vi "Load Config.vi"(8 "error in (no error)":errorcluster) -> (0 "error out":errorcluster, 3 "Array":T3(array[cluster]))   [LabVIEW 2019, in "LINX.lvlib" / "LINX.lvclass"]
uses:
  LINX.lvclass
  LINX Control Shortcut.ctl
  LINX Channel Type.ctl
  LINX Command Message.ctl
  <vilib>/Utility/config.llb/Read Key (String).vi
  <vilib>/Utility/config.llb/Read Key (I32).vi
  <vilib>/Utility/config.llb/NI_LVConfig.lvlib
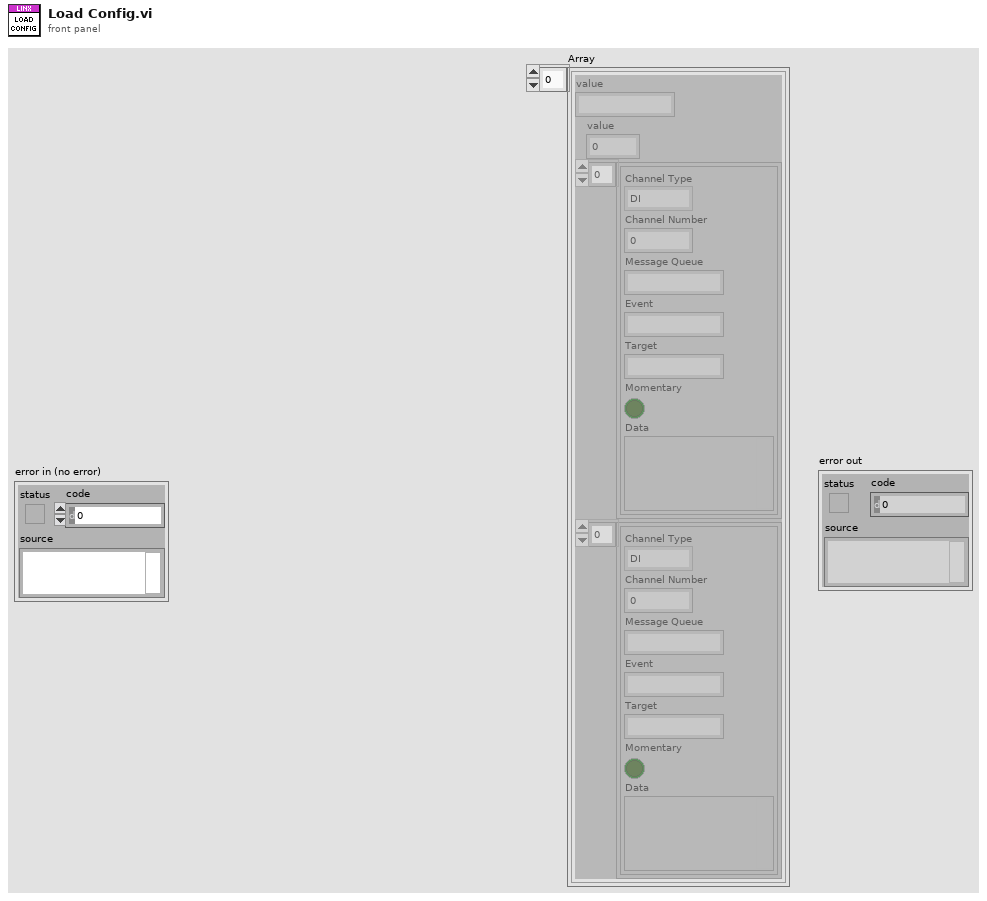
[diagram p1: front panel]
types:
  T1 = typedef "LINX.lvlib/LINX.lvclass/LINX Control Shortcut.ctl" = cluster{"Channel Type":T2, "Channel Number":u8, "Message Queue":string, "Event":string, "Target":string, "Momentary":bool, "Data":variant}
  T2 = typedef "LINX.lvlib/LINX.lvclass/LINX Channel Type.ctl" = enum16{"DI", "AI"}
  T3 = cluster{"value":string, "value":i32, T1[], T1[]}[]
  T4 = typedef "NI_LVConfig.lvlib/Config Data RefNum.ctl" = refnum<k1>
  T5 = typedef "LINX.lvlib/LINX.lvclass/LINX Command Message.ctl" = cluster{"Command":string, "Message Queue":string, "Event":string, "Target":string, "Momentary":bool, "Data":variant}
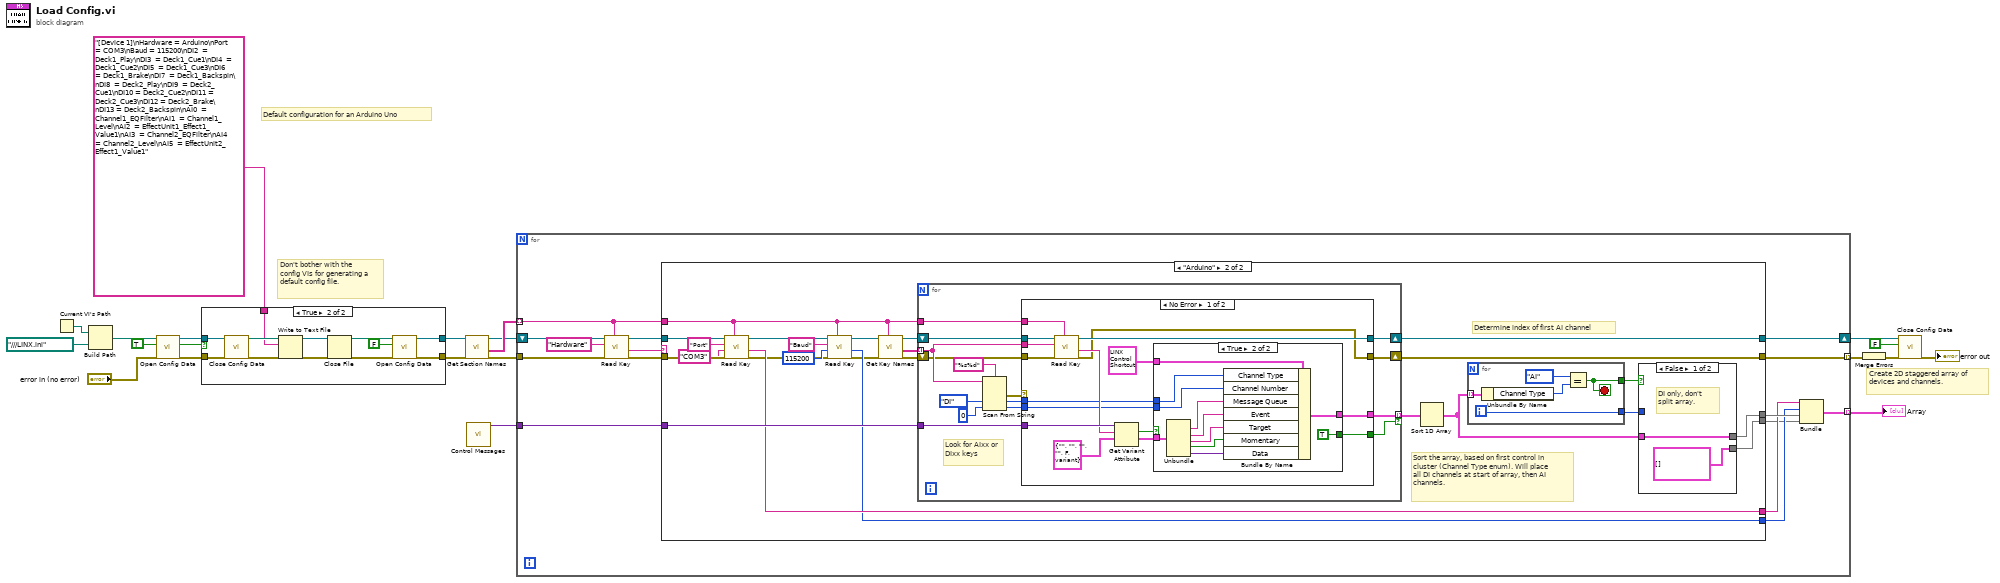
[diagram p0: block diagram]
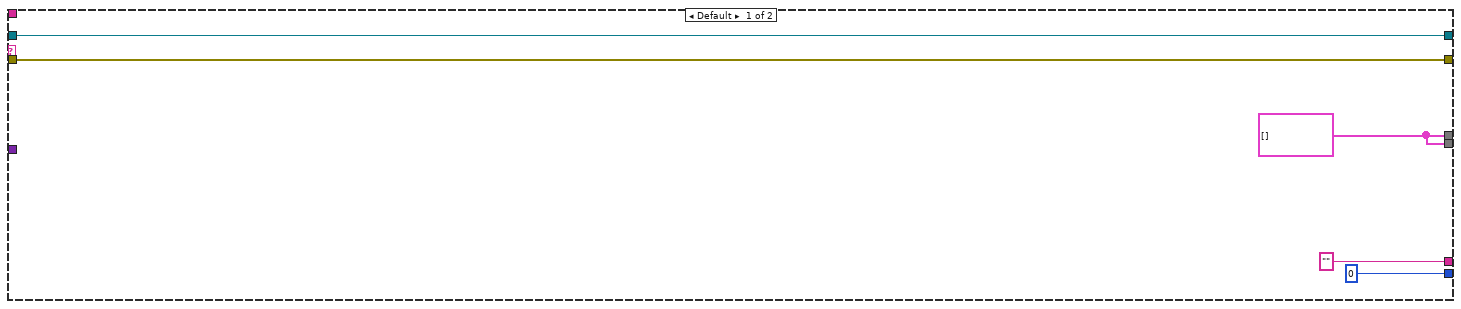
[diagram p3: hidden frame]
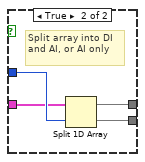
[diagram p4: hidden frame]
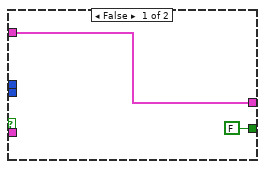
[diagram p5: hidden frame]
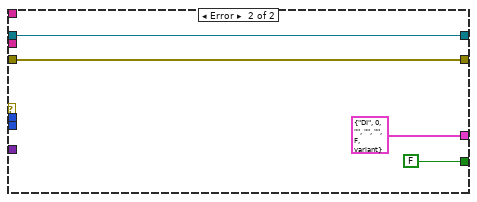
[diagram p6: hidden frame]
diagram:
  # "Don't bother with the config VIs for generating a default config file."
  # "Create 2D staggered array of devices and channels."
  # "Default configuration for an Arduino Uno"
  n1 = Current VI's Path() -> (path=w13:path)
  n2 = Build Path(base path=w13, name or relative path=path "../../../LINX.ini" ("configuration file path")) -> (appended path=w11:path)
  n3 = call <vilib>:"Open Config Data.vi"("error in (no error)"="error in (no error)", "create file if necessary (T)"=TRUE, "configuration file path"=w11) -> ("error out"=w6:errorcluster, "file created?"=w10:bool, "refnum"=w9:T4)  [unwired: 6 in]
  n4 = case shown="True" w10 {
    tunnel: w9 -> [w23 w35]
    tunnel: [w23 w24] -> w8
    tunnel: [w22 w25] -> w7
    tunnel: w6 -> [w22 w34]
    tunnel: "[Device 1]\nHardware = Arduino\nPort = COM3\nBaud = 115200\nDI2  = Deck1_Play\nDI3  = Deck1_Cue1\nDI4  = Deck1_Cue2\nDI5  = Deck1_Cue3\nDI6  = Deck1_Brake\nDI7  = Deck1_Backspin\nDI8  = Deck2_Play\nDI9  = Deck2_Cue1\nDI10 = Deck2_Cue2\nDI11 = Deck2_Cue3\nDI12 = Deck2_Brake\nDI13 = Deck2_Backspin\nAI0  = Channel1_EQFilter\nAI1  = Channel1_Level\nAI2  = EffectUnit1_Effect1_Value1\nAI3  = Channel2_EQFilter\nAI4  = Channel2_Level\nAI5  = EffectUnit2_Effect1_Value1" -> [_ w32]
    frame False {
    }
    frame True {
      n5 = call <vilib>:"Close Config Data.vi"("error in (no error)"=w34, "refnum"=w35) -> ("error out"=w31:errorcluster, "file path"=w33:path)  [unwired: 8 in]
      n6 = Write to Text File(file (use dialog)=w33, text=w32, error in=w31) -> (refnum out=w30:refnum<file>, error out=w29:errorcluster)  [unwired: 1 in, 1 out]
      n7 = Close File(refnum=w30, error in=w29) -> (path=w28:path, error out=w26:errorcluster)
      n8 = call <vilib>:"Open Config Data.vi"("error in (no error)"=w26, "create file if necessary (T)"=FALSE, "configuration file path"=w28) -> ("error out"=w25:errorcluster, "refnum"=w24:T4)  [unwired: 6 in, 1 out]
    }
  }
  n9 = call <vilib>:"Get Section Names.vi"("error in (no error)"=w7, "refnum"=w8) -> ("error out"=w17:errorcluster, "section names"=w19:string[], "refnum out"=w18:T4)  [unwired: 7 in]
  n10 = call "Control Messages.vi"() -> ("Shortcuts"=w20:variant)  [unwired: 11 in]
  n11 = for {
    tunnel: w19 -> [w46] mode=indexing
    tunnel: w17 -> [w38]
    shift-right: [w44] -> w15
    shift-left: w18 -> [w50]
    tunnel: w20 -> [w45]
    tunnel: [w42] -> w16 mode=indexing
    tunnel: [w36] -> w2 mode=indexing
    n12 = call-poly <vilib>:"Read Key.vi"("section"=w46, "error in (no error)"=w38, "key"="Hardware", "refnum"=w50) -> ("error out"=w37:errorcluster, "value"=w48:string, "refnum out"=w47:T4)  [unwired: 4 in, 1 out]
    n13 = case shown="\"Arduino\"" w48 {
      tunnel: w47 -> [w55 w80]
      tunnel: w46 -> [_ w73]
      tunnel: w45 -> [_ w72]
      tunnel: [w55 w70] -> w44
      tunnel: [w54 w64] -> w43
      tunnel: ["" ("value") w69] -> w41
      tunnel: [0 ("value") w68] -> w40
      tunnel: [w54 w63] -> w39
      tunnel: w37 -> [w51 w61]
      tunnel: [w51 w57] -> w36
      frame Default {
        w54 = T1[] []
      }
      frame "Arduino" {
        # "Determine index of first AI channel"
        # "Sort the array, based on first control in cluster (Channel Type enum). Will place all DI channels at start of array, then AI channels."
        n14 = call-poly <vilib>:"Read Key.vi"("section"=w73, "error in (no error)"=w61, "default value"="COM3", "key"="Port", "refnum"=w80) -> ("error out"=w59:errorcluster, "value"=w69:string, "refnum out"=w78:T4)  [unwired: 3 in, 1 out]
        n15 = call-poly <vilib>:"Read Key.vi"("section"=w73, "error in (no error)"=w59, "default value"=115200, "key"="Baud", "refnum"=w78) -> ("error out"=w58:errorcluster, "value"=w68:i32, "refnum out"=w76:T4)  [unwired: 3 in, 1 out]
        n16 = call <vilib>:"Get Key Names.vi"("section"=w73, "error in (no error)"=w58, "refnum"=w76) -> ("error out"=w56:errorcluster, "key names"=w75:string[], "refnum out"=w74:T4)  [unwired: 5 in, 1 out]
        n17 = for {
          tunnel: w75 -> [w103] mode=indexing
          shift-right: [w104] -> w70
          shift-left: w74 -> [w105]
          tunnel: w73 -> [w98]
          tunnel: w72 -> [w97]
          tunnel: [w95] -> w71 mode=indexing if=w94
          shift-right: [w93] -> w57
          shift-left: w56 -> [w92]
          # "Look for AIxx or DIxx keys"
          n18 = Scan From String(format string="%s%d", input string=w103, default 1=LINX_Channel_Type."DI" ("Channel Type"), default 2=u8 0 ("default value 2")) -> (error out=w101:errorcluster, output 1=w100:T2, output 2=w99:u8)  [unwired: 2 in, 2 out]
          n19 = case shown="No Error" w101 {
            tunnel: w105 -> [w122 w138]
            tunnel: [w121 w138] -> w104
            tunnel: w103 -> [w120 _]
            tunnel: w100 -> [w113 _]
            tunnel: w99 -> [w112 _]
            tunnel: w98 -> [w119 _]
            tunnel: w97 -> [w118 _]
            tunnel: [w111 T1 {"Channel Type"=enum."DI", "Channel Number"=0, "Message Queue"="", "Event"="", "Target"="", "Momentary"=FALSE, "Data"=variant} ("DAQmx Shortcut")] -> w95
            tunnel: [w110 FALSE] -> w94
            tunnel: w92 -> [w108 w136]
            tunnel: [w107 w136] -> w93
            frame No Error {
              n20 = call-poly <vilib>:"Read Key.vi"("section"=w119, "error in (no error)"=w108, "key"=w120, "refnum"=w122) -> ("error out"=w107:errorcluster, "value"=w117:string, "refnum out"=w121:T4)  [unwired: 4 in, 1 out]
              n21 = Get Variant Attribute(Variant=w118, name=w117, default value (empty Variant)=T5 {"Command"="", "Message Queue"="", "Event"="", "Target"="", "Momentary"=FALSE, "Data"=variant} ("LINX Command Message")) -> (found=w109:bool, value=w114:T5)  [unwired: 1 in, 2 out]
              n22 = case shown="True" w109 {
                tunnel: T1 {"Channel Type"=enum."AI", "Channel Number"=0, "Message Queue"="Mixer", "Event"="Value Change", "Target"="Crossfader", "Momentary"=FALSE, "Data"=variant} ("LINX Control Shortcut") -> [w124 w135]
                tunnel: w114 -> [_ w134]
                tunnel: w113 -> [_ w133]
                tunnel: w112 -> [_ w132]
                tunnel: [w124 w126] -> w111
                tunnel: [FALSE TRUE] -> w110
                frame False {
                }
                frame True {
                  n23 = Unbundle(w134) -> ("Message Queue"=w131:string, "Event"=w130:string, "Target"=w129:string, "Momentary"=w128:bool, "Data"=w127:variant)  [unwired: 1 out]
                  n24 = Bundle By Name(cluster=w135, "Channel Type"=w133, "Channel Number"=w132, "Message Queue"=w131, "Event"=w130, "Target"=w129, "Momentary"=w128, "Data"=w127) -> (w126:T1)
                }
              }
            }
            frame Error {
            }
          }
        }
        n25 = Sort 1D Array(array=w71) -> (sorted array=w65:T1[])
        n26 = for {
          tunnel: w65 -> [w88] mode=indexing
          tunnel: [w90] -> w66
          tunnel: [w89] -> w67
          i -> [w90]
          stop <- w89 stop-if-true
          n27 = Unbundle By Name(w88) -> ("Channel Type"=w87:T2)
          n28 = Equal?(x=LINX_Channel_Type."AI", y=w87) -> (x = y?=w89:bool)
        }
        n29 = case shown="False" w67 {
          tunnel: w66 -> [_ w86]
          tunnel: w65 -> [w82 w85]
          tunnel: [w82 w84] -> w64
          tunnel: [T1[] [] w83] -> w63
          frame False {
            # "DI only, don't split array."
          }
          frame True {
            # "Split array into DI and AI, or AI only"
            n30 = Split 1D Array(array=w85, index=w86) -> (first subarray=w84:T1[], second subarray=w83:T1[])
          }
        }
      }
    }
    n31 = Bundle("value"=w41, "value"=w40, w43, w39) -> (w42:cluster{"value":string, "value":i32, T1[], T1[]})  [unwired: 1 in]
  }
  "Array" <- w16
  n32 = Merge Errors(w2) -> (w1:errorcluster)
  n33 = call <vilib>:"Close Config Data.vi"("error in (no error)"=w1, "write file if changed (T)"=FALSE, "refnum"=w15) -> ("error out"=→"error out":errorcluster)  [unwired: 7 in, 1 out]
